vi "EventHandler.vi"(8 "error in (no error)":errorcluster, 11 "Navigator in":refnum<class "Navigator.lvclass">) -> (0 "error out":errorcluster, 3 "Navigator out":refnum<class "Navigator.lvclass">)   [LabVIEW 2024, in "Navigator.lvclass"]
doc: "Navigator event handling loop."
uses:
  Navigator.lvclass
  Navigator.lvclass/Navigator.ctl
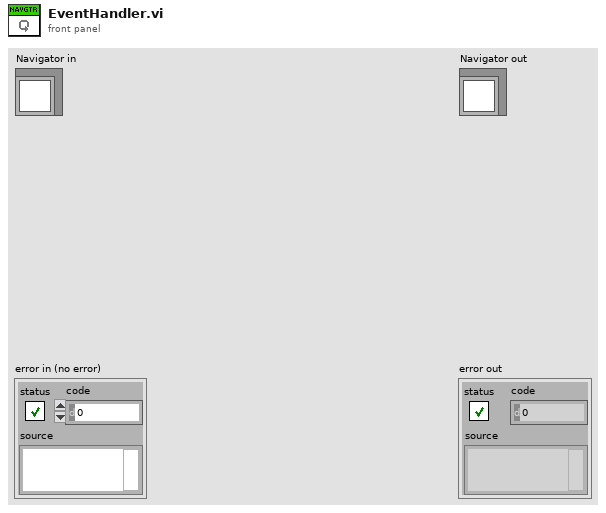
[diagram p1: front panel]
types:
  T1 = typedef "Navigator.lvclass/NavigatorEvents.ctl" = cluster{"go":refnum<user-event>, "push":refnum<user-event>, "pop":refnum<user-event>}
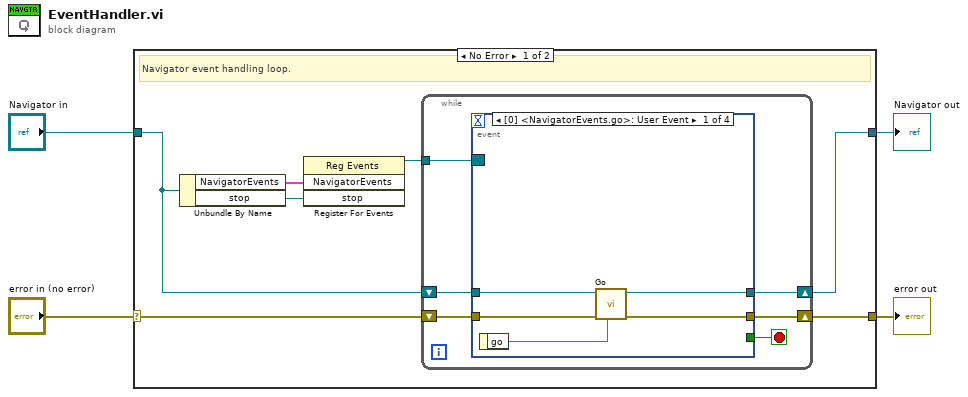
[diagram p0: block diagram]
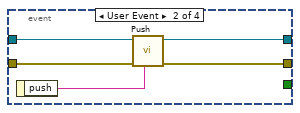
[diagram p2: hidden frame]
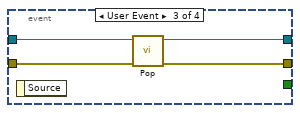
[diagram p3: hidden frame]
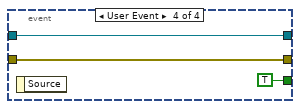
[diagram p4: hidden frame]
diagram:
  n1 = case shown="No Error" "error in (no error)" {
    selector: "error in (no error)" -> [w8 w36]
    tunnel: [w7 w36] -> w3
    tunnel: [w5 w35] -> w1
    tunnel: "Navigator in" -> [w6 w35]
    frame No Error {
      # "Navigator event handling loop."
      n2 = Unbundle By Name(w6) -> ("NavigatorEvents"=w10:T1, "stop"=w9:refnum<user-event>)
      n3 = register-events(w10, w9) -> (reference out=w11:refnum<event-registration>)  [unwired: 2 in, 1 out]
      n4 = while {
        tunnel: w11 -> [w17]
        shift-right: [w15] -> w7
        shift-left: w8 -> [w16]
        shift-right: [w13] -> w5
        shift-left: w6 -> [w14]
        stop <- w12 stop-if-true
        n5 = event shown="[0] <NavigatorEvents.go>: User Event" {
          selector: w17 -> [_ _ _ _]
          dyn-events: _ -> [_ _ _ _]
          timeout: _ -> [_ _ _ _]
          tunnel: w16 -> [w21 w26 w28 w34]
          tunnel: [w19 w24 w29 w34] -> w15
          tunnel: w14 -> [w22 w27 w31 w33]
          tunnel: [w20 w25 w30 w33] -> w13
          tunnel: [_ _ _ TRUE] -> w12
          event User Event {
            n6 = event-data() -> ("go"=w18:string)  [unwired: 1 in]
            n7 = call "Go.vi"("Route"=w18, "error in (no error)"=w21, "Navigator in"=w22) -> ("error out"=w19:errorcluster, "Navigator out"=w20:refnum<class "Navigator.lvclass">)  [unwired: 7 in]
          }
          event User Event {
            n8 = event-data() -> ("push"=w23:string)  [unwired: 1 in]
            n9 = call "Push.vi"("Route"=w23, "error in (no error)"=w26, "Navigator in"=w27) -> ("error out"=w24:errorcluster, "Navigator out"=w25:refnum<class "Navigator.lvclass">)  [unwired: 7 in]
          }
          event User Event {
            n10 = event-data() -> ()  [unwired: 1 in, 1 out]
            n11 = call "Pop.vi"("error in (no error)"=w28, "Navigator in"=w31) -> ("error out"=w29:errorcluster, "Navigator out"=w30:refnum<class "Navigator.lvclass">)  [unwired: 8 in]
          }
          event User Event {
            n12 = event-data() -> ()  [unwired: 1 in, 1 out]
          }
        }
      }
    }
    frame Error {
    }
  }
  "error out" <- w3
  "Navigator out" <- w1
